vi "Modbus Slave Write Server Register.vi"() -> ()   [LabVIEW 2021]
uses:
  <vilib>/Utility/file.llb/Read Delimited Spreadsheet (string).vi
  <vilib>/NI/Modbus Library/API/Wrapper/Create TCP Slave.vi
  <vilib>/NI/Modbus Library/API/Slave/Modbus Slave.lvclass
  <vilib>/NI/Modbus Library/API/Wrapper/API Main.lvlib
panel:
  out "error out":errorcluster
  in  "stop":bool
  out "Array 2":u16[](array[numeric])
  out "Numeric":i32
  out "Array":u16[](array[numeric])
  in  "Table Control":string[][](table)
  out "all rows":string[][](array[string])
  in  "file path (dialog if empty)":path
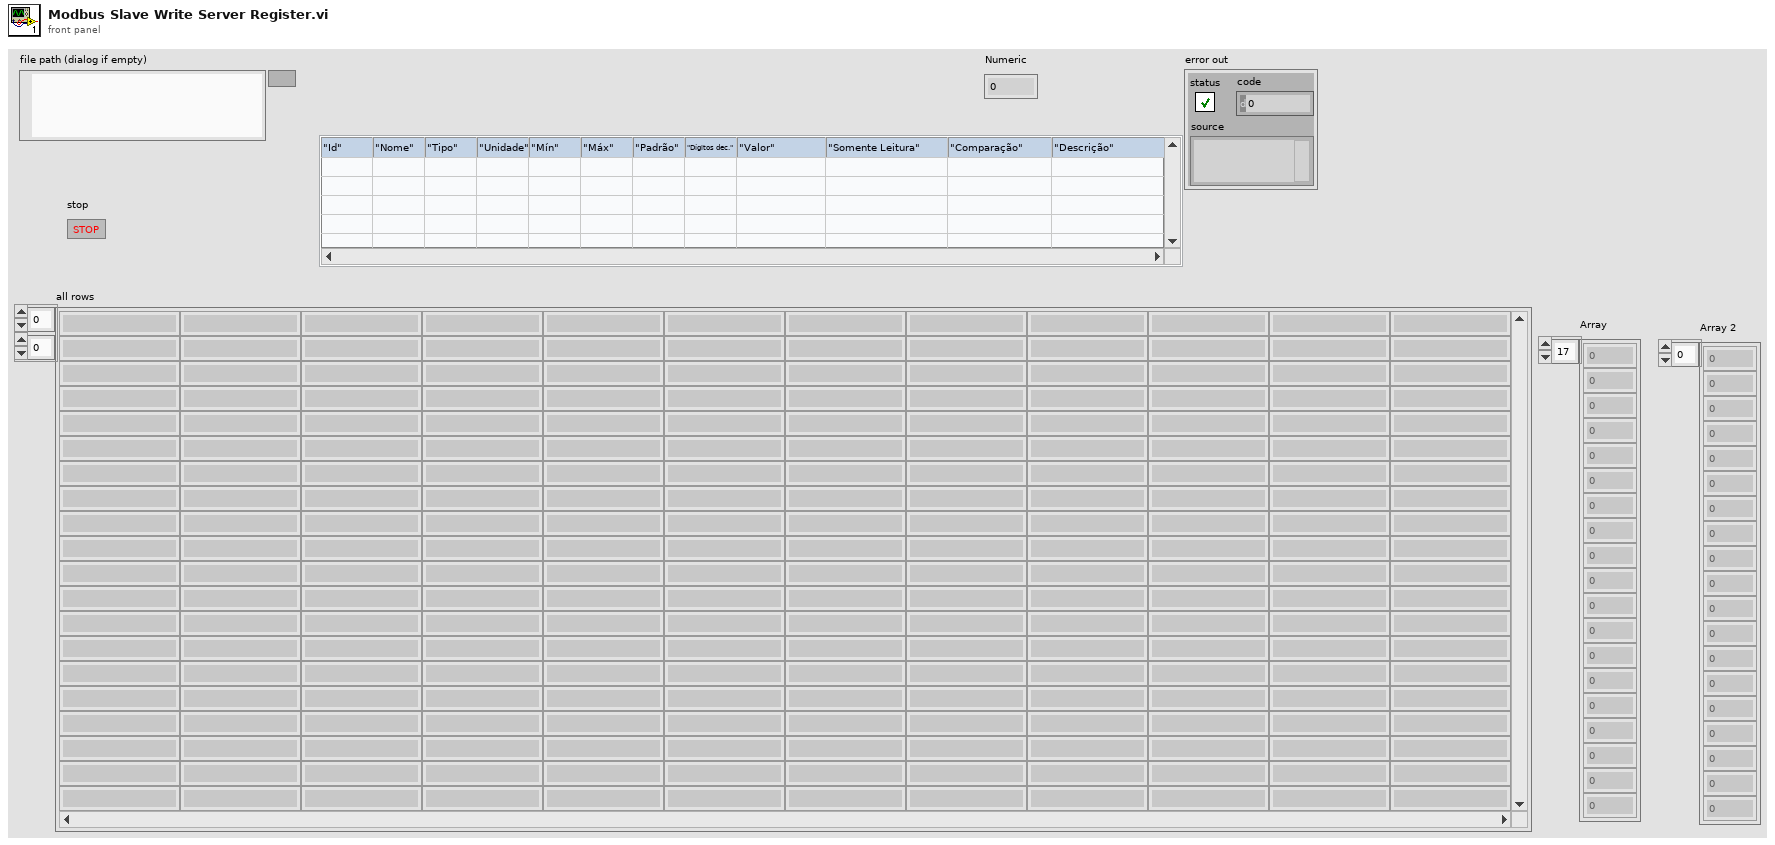
[diagram p1: front panel]
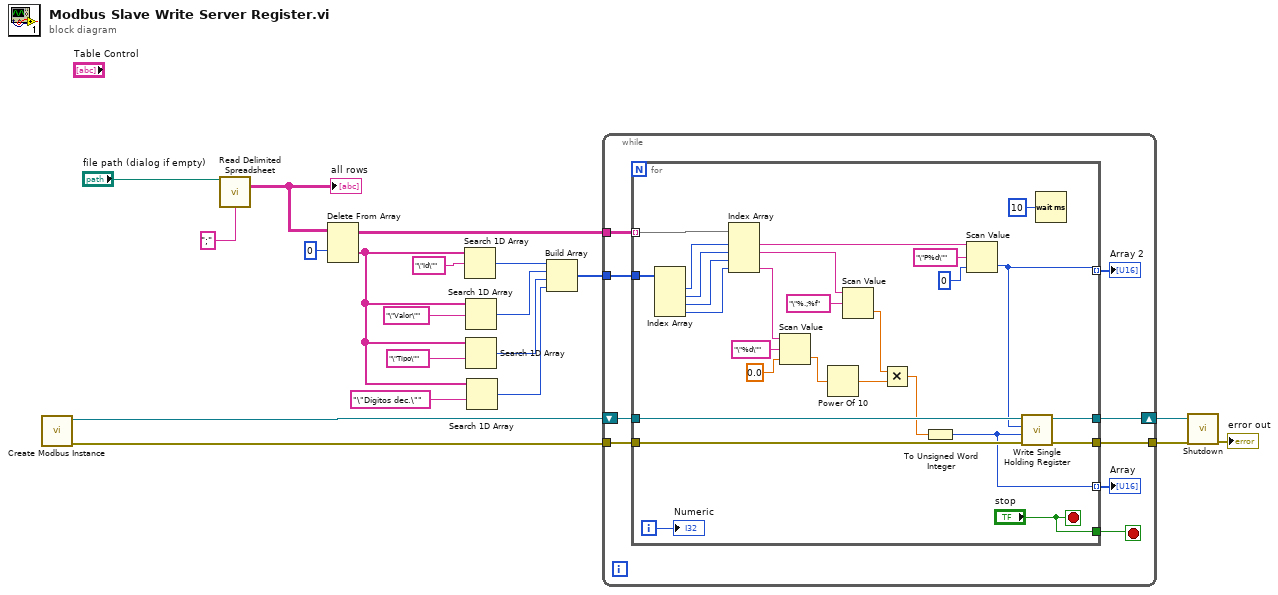
[diagram p0: block diagram]
diagram:
  n1 = call-poly <vilib>:"Create Modbus Instance.vi"() -> ("error out"=w15:errorcluster, "TCP slave instance"=w16:refnum<class "Modbus Slave.lvclass">)  [unwired: 10 in]
  n2 = call-poly <vilib>:"Read Delimited Spreadsheet.vi"("file path (dialog if empty)"="file path (dialog if empty)", "delimiter (\\t)"=";" ("delimiter (\\t)")) -> ("all rows"=w18:string[][])  [unwired: 8 in, 5 out]
  "all rows" <- w18
  n3 = Delete From Array(array=w18, index (row)=0) -> (deleted portion=w10:string[], array with subset deleted=w9:string[][])  [unwired: 2 in]
  n4 = Search 1D Array(1D array=w10, element="\"Id\"") -> (index of element=w6:i32)  [unwired: 1 in]
  n5 = Search 1D Array(1D array=w10, element="\"Valor\"") -> (index of element=w5:i32)  [unwired: 1 in]
  n6 = Search 1D Array(1D array=w10, element="\"Tipo\"") -> (index of element=w4:i32)  [unwired: 1 in]
  n7 = Search 1D Array(1D array=w10, element="\"Dígitos dec.\"") -> (index of element=w3:i32)  [unwired: 1 in]
  n8 = Build Array(w6, w5, w4, w3) -> (w2:i32[])
  n9 = while {
    tunnel: w9 -> [w27]
    tunnel: w2 -> [w24]
    shift-right: [w26] -> w8
    shift-left: w16 -> [w29]
    tunnel: w15 -> [w28]
    tunnel: [w25] -> w7
    stop <- w21 stop-if-true
    n10 = for {
      tunnel: w29 -> [w56]
      tunnel: w28 -> [w55]
      tunnel: w27 -> [w50] mode=indexing
      tunnel: [w54] -> w26
      tunnel: [w53] -> w25
      tunnel: w24 -> [w52]
      tunnel: [w34] -> w23 mode=indexing
      tunnel: [w31] -> w22 mode=indexing
      tunnel: ["stop"] -> w21
      i -> [w32]
      stop <- "stop" stop-if-true
      n11 = Index Array(array=w52) -> (element #1=w51:i32, element #2=w46:i32, element #3=w45:i32, element #4=w44:i32)  [unwired: 4 in]
      n12 = Index Array(array=w50, index #1=w51, index #2=w46, index #3=w45, index #4=w44) -> (element #1=w49:string, element #2=w36:string, element #4=w41:string)  [unwired: 1 out]
      n13 = Scan Value(string=w41, format string="\"%d\"", default (0 dbl)=0.0 ("default value 1")) -> (value=w40:dbl)  [unwired: 1 out]
      n14 = Power Of 10(x=w40) -> (10^x=w39:dbl)
      n15 = Scan Value(string=w36, format string="\"%.;%f") -> (value=w35:dbl)  [unwired: 1 in, 1 out]
      n16 = Multiply(x=w35, y=w39) -> (x*y=w38:dbl)
      n17 = To Unsigned Word Integer(number=w38) -> (unsigned 16bit integer=w34:u16)
      n18 = Scan Value(string=w49, format string="\"P%d\"", default (0 dbl)=u16 0 ("default value 1")) -> (value=w31:u16)  [unwired: 1 out]
      n19 = call-dynamic "Write Single Holding Register.vi"("error in"=w55, "register to write"=w34, "address"=w31, "Modbus slave in"=w56) -> ("error out"=w53:errorcluster, "Modbus slave out"=w54:refnum<class "Modbus Slave.lvclass">)  [unwired: 6 in]
      n20 = Wait (ms)(milliseconds to wait=u32 10) -> ()  [unwired: 1 out]
      "Numeric" <- w32
    }
    "Array" <- w23
    "Array 2" <- w22
  }
  n21 = call-dynamic "Shutdown.vi"("error in"=w7, "Modbus slave in"=w8) -> ("error out"=→"error out":errorcluster)  [unwired: 9 in]
